vi "test_BuildAssets.vi"() -> (3 "Pass?":bool)   [LabVIEW 2019, in "Tests.SolutionBuilder.lvlib"]
uses:
  Tests.SolutionBuilder.lvlib
  SolutionBuilder/SolutionBuilder.lvclass
  SolutionBuilder/BuildManager/GeneratedFile.ctl
  SolutionBuilder/BuildManager/BuildManager.lvclass
panel:
  out "Result paths":path[](array[path])
  out "error out":errorcluster
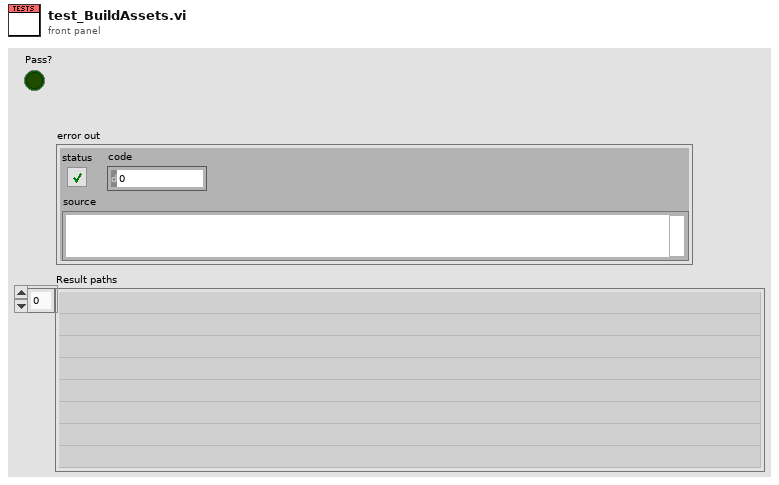
[diagram p1: front panel]
types:
  T1 = typedef "SolutionBuilder.lvlib/BuildManager.lvclass/GeneratedFile.ctl" = map{cluster{"Project path":string, "Build spec name":string}, set{string}}
  T2 = typedef "SolutionBuilder.lvlib/BuildManager.lvclass/BuildProjectInfo.ctl" = cluster{"Project path":string, "Build spec name":string, "Target":string, "Version string":string}
  T3 = typedef "SolutionBuilder.lvlib/SolutionBuilder.lvclass/NamePathMap.ctl" = map{string, path}
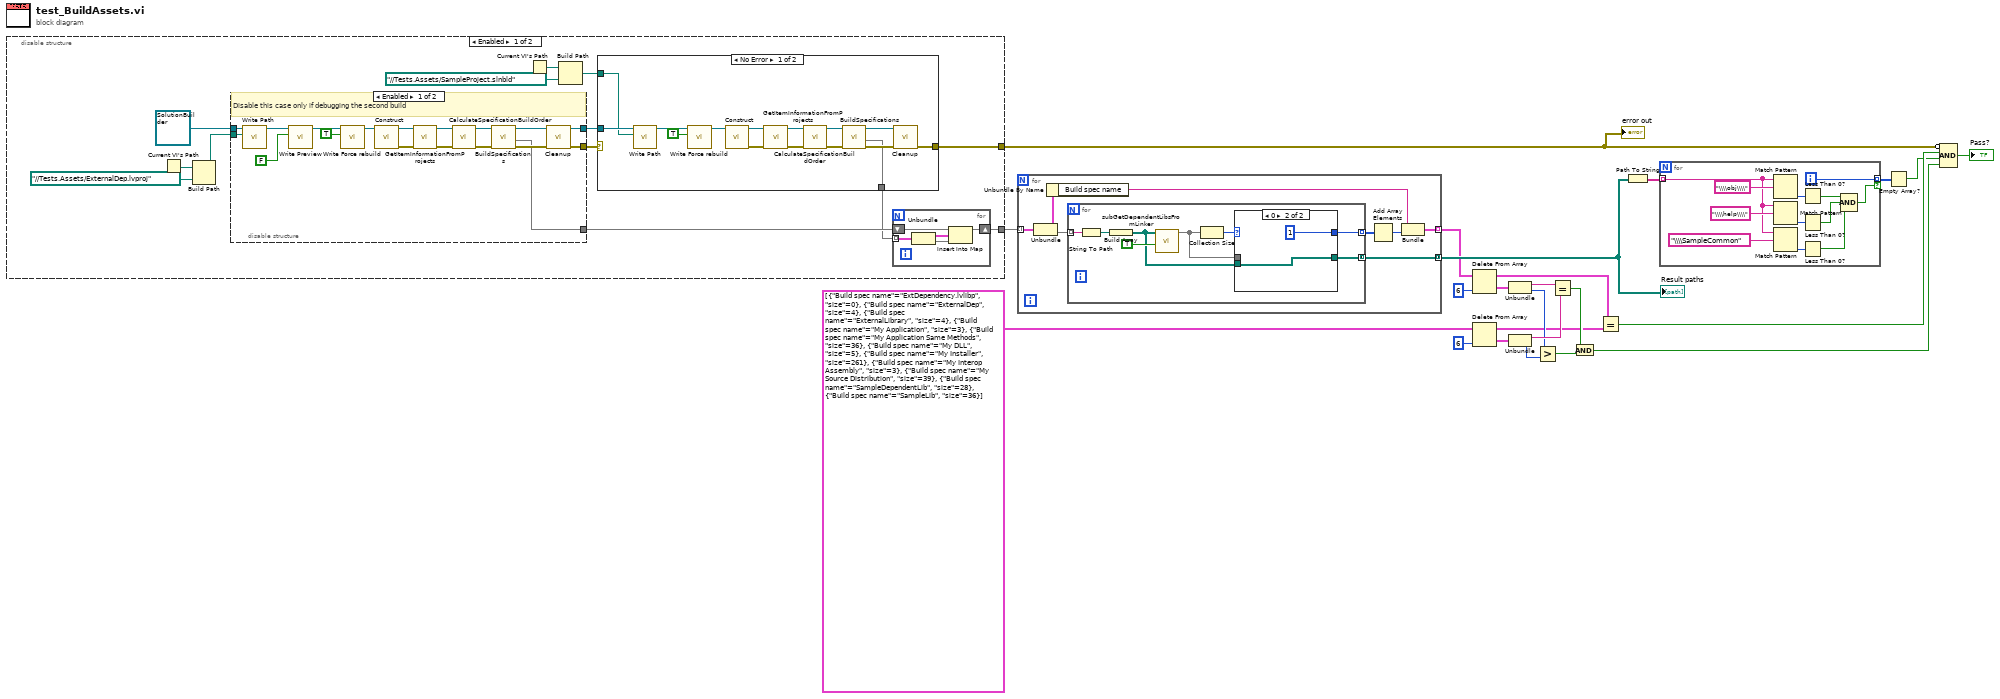
[diagram p0: block diagram]
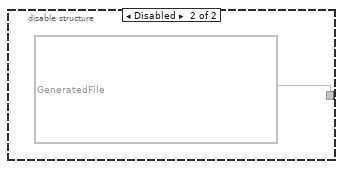
[diagram p4: hidden frame]
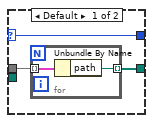
[diagram p5: hidden frame]
diagram:
  n1 = disable-structure shown="Enabled" {
    disable-tunnel: [w36 _] -> w23
    disable-tunnel: [w24 T1 data[36679B] ("Generated file")] -> w20
    frame Enabled {
      n2 = Current VI's Path() -> (path=w34:path)
      n3 = Build Path(base path=w34, name or relative path=path "../../Tests.Assets/ExternalDep.lvproj" ("Path")) -> (appended path=w32:path)
      n4 = disable-structure shown="Enabled" {
        disable-tunnel: refnum<class "SolutionBuilder.lvclass"> refnum ("SolutionBuilder in") -> [w59 w60]
        disable-tunnel: w32 -> [w55 _]
        disable-tunnel: [w51 w60] -> w31
        disable-tunnel: [w49 _] -> w30
        disable-tunnel: [w48 _] -> w26
        frame Enabled {
          # "Disable this case only if debugging the second build"
          n5 = call "Write Path.vi"("Path"=w55, "SolutionBuilder in"=w59) -> ("SolutionBuilder out"=w46:refnum<class "SolutionBuilder.lvclass">)  [unwired: 9 in]
          n6 = call "Write Preview.vi"("Preview?"=FALSE, "SolutionBuilder in"=w46) -> ("SolutionBuilder out"=w44:refnum<class "SolutionBuilder.lvclass">)  [unwired: 9 in]
          n7 = call "Write Force rebuild.vi"("Force rebuild"=TRUE, "SolutionBuilder in"=w44) -> ("SolutionBuilder out"=w43:refnum<class "SolutionBuilder.lvclass">)  [unwired: 9 in]
          n8 = call "Construct.vi"("SolutionBuilder in"=w43) -> ("error out"=w54:errorcluster, "SolutionBuilder out"=w58:refnum<class "SolutionBuilder.lvclass">)  [unwired: 9 in]
          n9 = call "GetItemInformationFromProjects.vi"("error in (no error)"=w54, "SolutionBuilder in"=w58) -> ("error out"=w53:errorcluster, "SolutionBuilder out"=w57:refnum<class "SolutionBuilder.lvclass">)  [unwired: 8 in]
          n10 = call "CalculateSpecificationBuildOrder.vi"("error in (no error)"=w53, "SolutionBuilder in"=w57) -> ("error out"=w52:errorcluster, "SolutionBuilder out"=w56:refnum<class "SolutionBuilder.lvclass">)  [unwired: 8 in]
          n11 = call "BuildSpecifications.vi"("error in (no error)"=w52, "SolutionBuilder in"=w56) -> ("error out"=w50:errorcluster, "Generated file"=w48:T1, "SolutionBuilder out"=w47:refnum<class "SolutionBuilder.lvclass">)  [unwired: 7 in]
          n12 = call "Cleanup.vi"("error in (no error)"=w50, "SolutionBuilder in"=w47) -> ("error out"=w49:errorcluster, "SolutionBuilder out"=w51:refnum<class "SolutionBuilder.lvclass">)  [unwired: 8 in]
        }
        frame Disabled {
        }
      }
      n13 = Current VI's Path() -> (path=w29:path)
      n14 = Build Path(base path=w29, name or relative path=path "../../Tests.Assets/SampleProject.slnbld" ("Path")) -> (appended path=w27:path)
      n15 = case shown="No Error" w30 {
        selector: w30 -> [_ w76]
        tunnel: w31 -> [w69 _]
        tunnel: [w67 w76] -> w36
        tunnel: w27 -> [w66 _]
        tunnel: [w65 _] -> w25
        frame No Error {
          n16 = call "Write Path.vi"("Path"=w66, "SolutionBuilder in"=w69) -> ("SolutionBuilder out"=w62:refnum<class "SolutionBuilder.lvclass">)  [unwired: 9 in]
          n17 = call "Write Force rebuild.vi"("Force rebuild"=TRUE, "SolutionBuilder in"=w62) -> ("SolutionBuilder out"=w61:refnum<class "SolutionBuilder.lvclass">)  [unwired: 9 in]
          n18 = call "Construct.vi"("SolutionBuilder in"=w61) -> ("error out"=w73:errorcluster, "SolutionBuilder out"=w70:refnum<class "SolutionBuilder.lvclass">)  [unwired: 9 in]
          n19 = call "GetItemInformationFromProjects.vi"("error in (no error)"=w73, "SolutionBuilder in"=w70) -> ("error out"=w74:errorcluster, "SolutionBuilder out"=w71:refnum<class "SolutionBuilder.lvclass">)  [unwired: 8 in]
          n20 = call "CalculateSpecificationBuildOrder.vi"("error in (no error)"=w74, "SolutionBuilder in"=w71) -> ("error out"=w75:errorcluster, "SolutionBuilder out"=w72:refnum<class "SolutionBuilder.lvclass">)  [unwired: 8 in]
          n21 = call "BuildSpecifications.vi"("error in (no error)"=w75, "SolutionBuilder in"=w72) -> ("error out"=w68:errorcluster, "Generated file"=w65:T1, "SolutionBuilder out"=w64:refnum<class "SolutionBuilder.lvclass">)  [unwired: 7 in]
          n22 = call "Cleanup.vi"("error in (no error)"=w68, "SolutionBuilder in"=w64) -> ("error out"=w67:errorcluster)  [unwired: 8 in, 1 out]
        }
        frame Error {
        }
      }
      n23 = for {
        shift-right: [w37] -> w24
        shift-left: w26 -> [w40]
        tunnel: w25 -> [w41] mode=indexing
        n24 = Unbundle(w41) -> ("Parent info"=w39:T2, "Generated files"=w38:set{string})
        n25 = Insert Into Map(map in=w40, key=w39, value=w38) -> (map out=w37:T1)  [unwired: 2 out]
      }
    }
    frame Disabled {
    }
  }
  "error out" <- w23
  n26 = for {
    tunnel: w20 -> [w85] mode=indexing
    tunnel: [w79] -> w5 mode=indexing
    tunnel: [w78] -> w19 mode=concatenating
    n27 = Unbundle(w85) -> ("Parent info"=w84:T2, "Generated files"=w83:set{string})
    n28 = Unbundle By Name(w84) -> ("Build spec name"=w81:string)
    n29 = for {
      tunnel: w83 -> [w92] mode=indexing
      tunnel: [w87] -> w82 mode=indexing
      tunnel: [w89] -> w78 mode=concatenating
      n30 = String To Path(string=w92) -> (path=w91:path)
      n31 = Build Array(w91) -> (w86:path[])
      n32 = call "subGetDependentLibsFromLinker.vi"("All?"=TRUE, "Paths"=w86) -> ("Dependency libs"=w90:T3)  [unwired: 8 in, 1 out]
      n33 = Collection Size(1:w90) -> (0:w88:i32)
      n34 = case shown="0" w88 {
        selector: w88 -> [w94 _]
        tunnel: w90 -> [w96 _]
        tunnel: [w95 w100] -> w89
        tunnel: [w94 1 ("size")] -> w87
        tunnel: w86 -> [_ w100]
        frame Default {
          n35 = for {
            tunnel: w96 -> [w98] mode=indexing
            tunnel: [w97] -> w95 mode=indexing
            n36 = Unbundle By Name(w98) -> ("path"=w97:path)
          }
        }
        frame 0 {
        }
      }
    }
    n37 = Add Array Elements(numeric array=w82) -> (sum=w80:i32)
    n38 = Bundle("Build spec name"=w81, "size"=w80) -> (w79:cluster{"Build spec name":string, "size":i32})  [unwired: 1 in]
  }
  "Result paths" <- w19
  n39 = Delete From Array(array=w5, index=6) -> (deleted portion=w13:cluster{"Build spec name":string, "size":i32}, array with subset deleted=w4:cluster{"Build spec name":string, "size":i32}[])  [unwired: 1 in]
  n40 = Delete From Array(array=cluster{"Build spec name":string, "size":i32}[] [{"Build spec name"="ExtDependency.lvlibp", "size"=0}, {"Build spec name"="ExternalDep", "size"=4}, {"Build spec name"="ExternalLibrary", "size"=4}, {"Build spec name"="My Application", "size"=3}, {"Build spec name"="My Application Same Methods", "size"=36}, {"Build spec name"="My DLL", "size"=5}, {"Build spec name"="My Installer", "size"=261}, {"Build spec name"="My Interop Assembly", "size"=3}, {"Build spec name"="My Source Distribution", "size"=39}, {"Build spec name"="SampleDependentLib", "size"=28}, {"Build spec name"="SampleLib", "size"=36}] ("Array"), index=6) -> (deleted portion=w12:cluster{"Build spec name":string, "size":i32}, array with subset deleted=w2:cluster{"Build spec name":string, "size":i32}[])  [unwired: 1 in]
  n41 = Unbundle(w13) -> ("Build spec name"=w11:string, "size"=w9:i32)
  n42 = Unbundle(w12) -> ("Build spec name"=w10:string, "size"=w8:i32)
  n43 = Greater?(x=w9, y=w8) -> (0:w6:bool)
  n44 = Equal?(x=w11, y=w10) -> (x = y?=w7:bool)
  n45 = And(x=w7, y=w6) -> (x .and. y?=w1:bool)
  n46 = Equal?(x=w4, y=w2) -> (x = y?=w18:bool)
  n47 = Path To String(path=w19) -> (string=w21:string[])
  n48 = for {
    tunnel: w21 -> [w102] mode=indexing
    tunnel: [w110] -> w17 mode=indexing if=w105
    i -> [w110]
    n49 = Match Pattern(string=w102, regular expression="\\\\obj\\\\") -> (offset past match=w111:i32)  [unwired: 1 in, 3 out]
    n50 = Match Pattern(string=w102, regular expression="\\\\help\\\\") -> (offset past match=w109:i32)  [unwired: 1 in, 3 out]
    n51 = Match Pattern(string=w102, regular expression="\\\\SampleCommon") -> (offset past match=w103:i32)  [unwired: 1 in, 3 out]
    n52 = Less Than 0?(x=w111) -> (x < 0?=w106:bool)
    n53 = Less Than 0?(x=w109) -> (x < 0?=w107:bool)
    n54 = Less Than 0?(x=w103) -> (x < 0?=w101:bool)
    n55 = Compound Arithmetic op=AND(w106, w107, w101) -> (w105:bool)
  }
  n56 = Empty Array?(array=w17) -> (empty?=w16:bool)
  n57 = Compound Arithmetic op=AND(invert w23, w18, w16, w1) -> (→"Pass?":bool)
